vi "SeqEditor_Allseqlist-menu.vi"(8 "error in (no error)":errorcluster, 10 "String":string, 11 "NLTest in":refnum<class "NLTest.lvclass">) -> (0 "error out":errorcluster, 3 "NLTest out":refnum<class "NLTest.lvclass">)   [LabVIEW 2017, in "NLTest.lvclass"]
uses:
  NLTest.lvclass
  NLTest.lvclass/NLTest.ctl
  allseqanddata.ctl
panel:
  in  "确认":bool
  in  "新名称":string
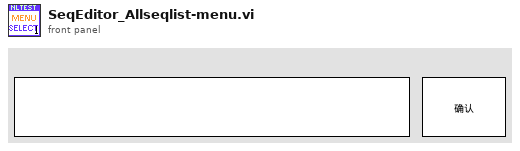
[diagram p1: front panel]
types:
  T1 = enum32{"Invalid", "Standard", "Closed", "Hidden", "Minimized", "Maximized"}
  T2 = typedef "NLTest.lvclass/allseqanddata.ctl" = cluster{"seqname":string, "seqdata":string[]}
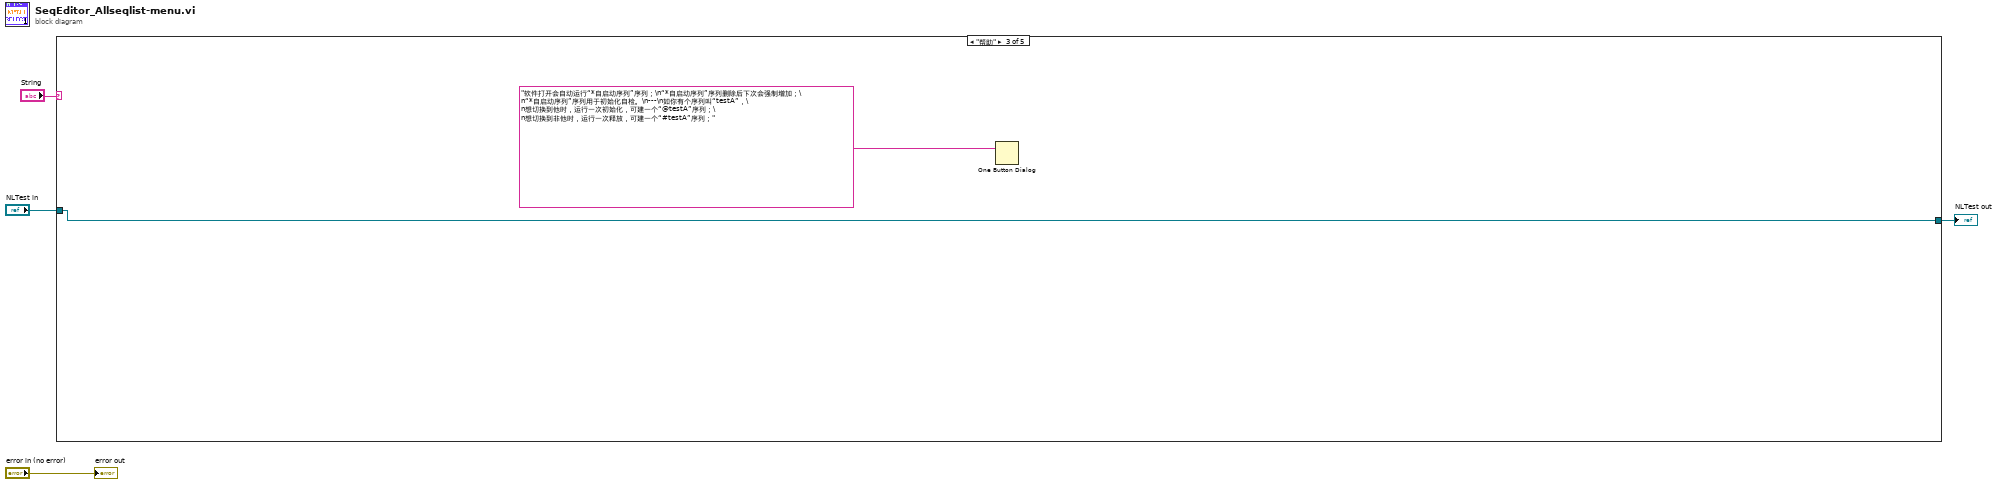
[diagram p0: block diagram]
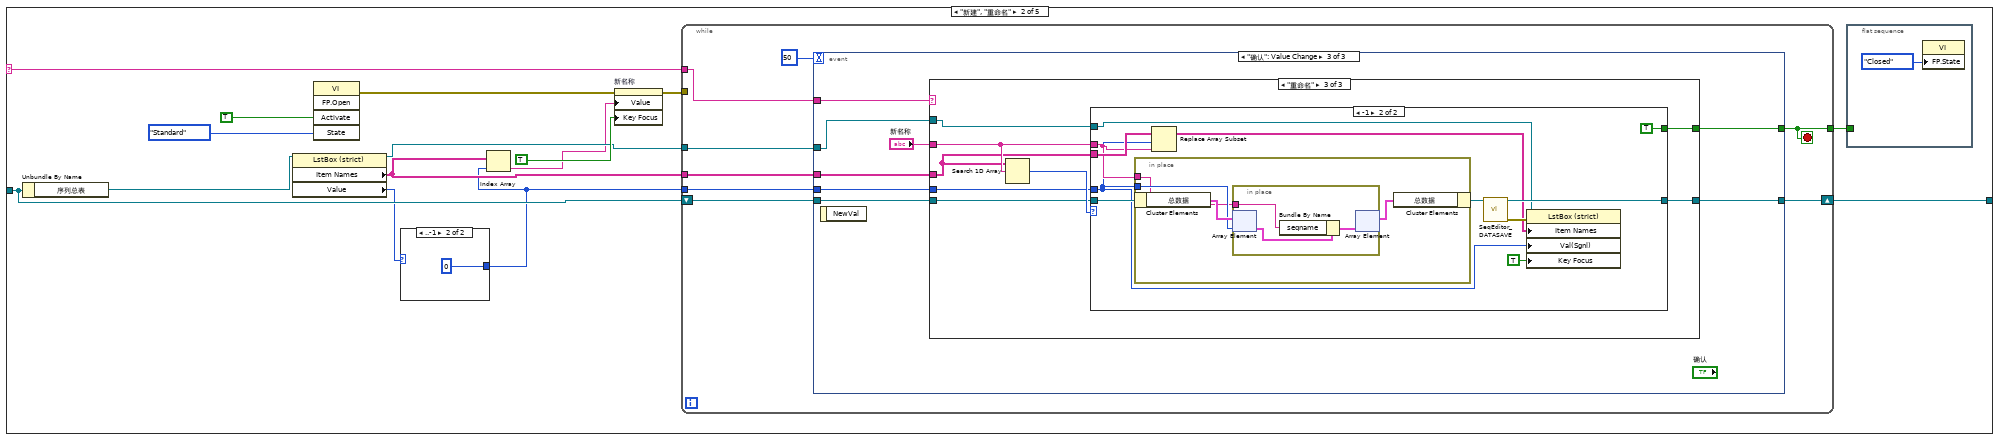
[diagram p3: hidden frame]
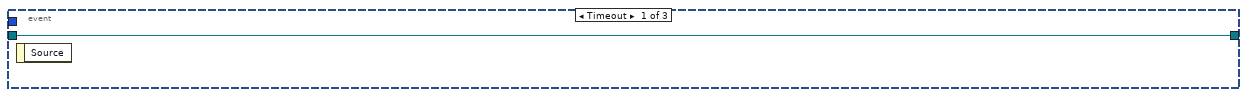
[diagram p5: hidden frame]
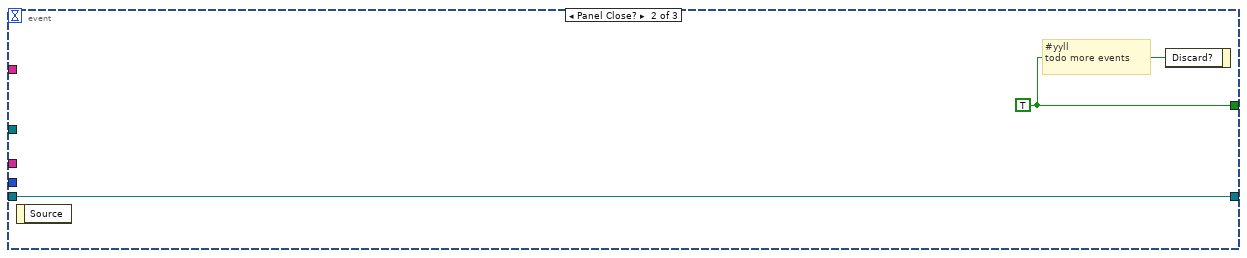
[diagram p6: hidden frame]
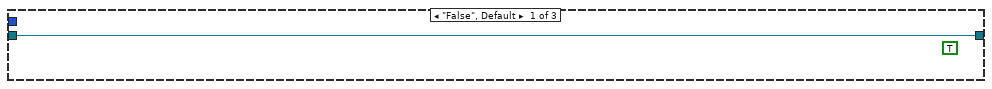
[diagram p7: hidden frame]
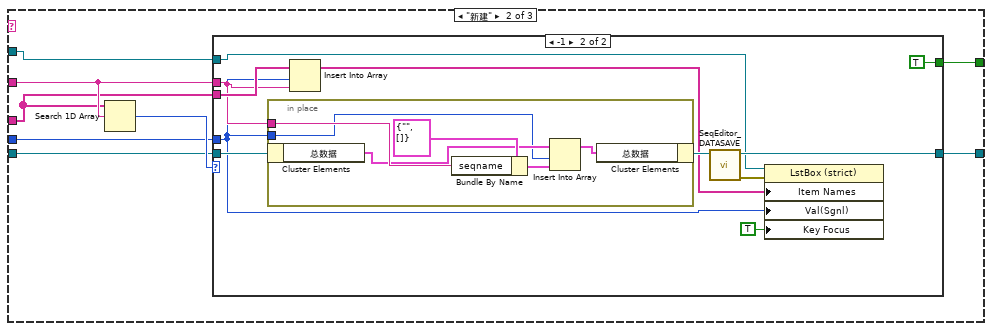
[diagram p8: hidden frame]
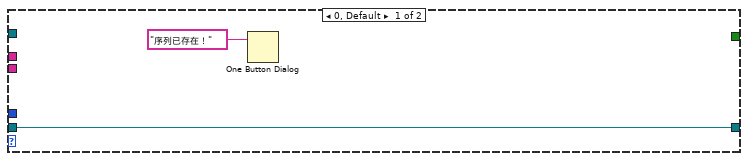
[diagram p9: hidden frame]
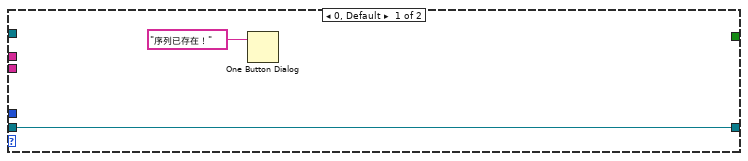
[diagram p10: hidden frame]
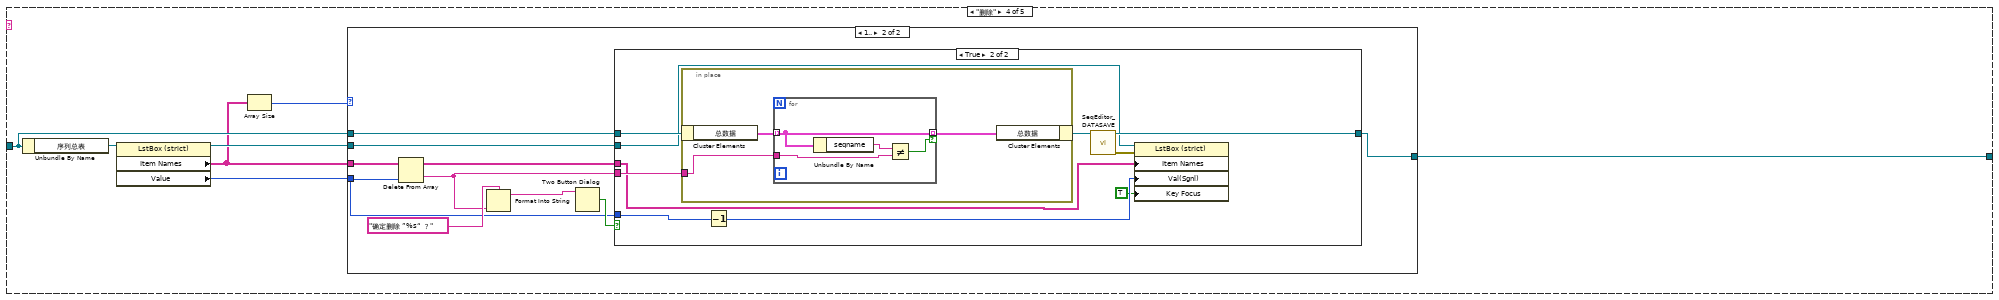
[diagram p11: hidden frame]
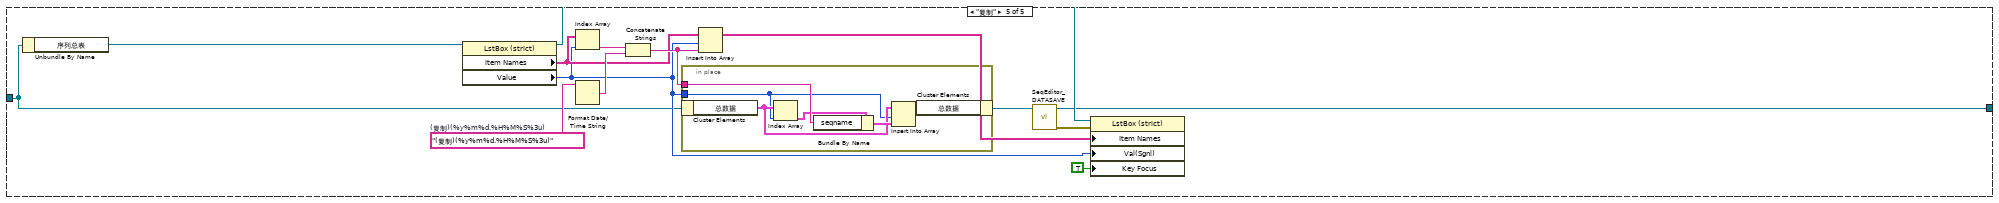
[diagram p14: hidden frame]
diagram:
  n1 = case shown="\"帮助\"" "String" {
    selector: "String" -> [_ w11 _ _ _]
    tunnel: "NLTest in" -> [w5 w14 w99 w105 w139]
    tunnel: [w5 w10 w99 w106 w138] -> w1
    frame Default {
    }
    frame "新建", "重命名" {
      n2 = Unbundle By Name(w14) -> ("序列总表"=w13:refnum<vi>)
      n3 = property class="LstBox (strict)"(reference=w13) -> (reference out=w9:refnum<vi>, "Item Names"=w12:string[], "Value"=w7:i32)  [unwired: 1 in, 1 out]
      n4 = invoke class="VI" method="FP.Open"("Activate"=TRUE ("Activate?"), "State"=T1."Standard") -> (error out=w19:errorcluster)  [unwired: 3 in, 4 out]
      n5 = case shown="..-1" w7 {
        selector: w7 -> [w21 _]
        tunnel: [w21 0] -> w6
        frame 0, Default {
        }
        frame ..-1 {
        }
      }
      n6 = Index Array(array=w12, index=w6) -> (element=w8:string)
      n7 = property on="新名称" class="Str"(error in=w19, "Value"=w8, "Key Focus"=TRUE) -> (error out=w18:errorcluster)  [unwired: 1 in, 1 out]
      n8 = while {
        tunnel: [w29] -> w15
        tunnel: w18 -> [_]
        tunnel: w11 -> [w30]
        tunnel: w12 -> [w27]
        tunnel: w9 -> [w25]
        tunnel: w6 -> [w24]
        shift-right: [w26] -> w10
        shift-left: w14 -> [w28]
        stop <- w29 stop-if-true
        n9 = event shown="[2] \"确认\": Value Change" {
          selector: _ -> [_ _ _]
          dyn-events: _ -> [_ _ _]
          timeout: 50 -> [_ _ _]
          tunnel: w30 -> [_ _ w42]
          tunnel: [_ w34 w35] -> w29
          tunnel: w28 -> [w32 w33 w41]
          tunnel: w27 -> [_ _ w39]
          tunnel: [w32 w33 w38] -> w26
          tunnel: w25 -> [_ _ w37]
          tunnel: w24 -> [_ _ w36]
          event Timeout {
            n10 = event-data() -> ()  [unwired: 1 in, 1 out]
          }
          event Panel Close? {
            w34 = TRUE ("Discard?")
            # "#yyll\ntodo more events"
            n11 = event-data() -> ()  [unwired: 1 in, 1 out]
            n12 = event-data("Discard?"=w34) -> ()  [unwired: 1 in, 1 out]
          }
          event "确认": Value Change {
            n13 = event-data() -> ()  [unwired: 1 in, 1 out]
            n14 = case shown="\"重命名\"" w42 {
              tunnel: w41 -> [w43 w50 w77]
              tunnel: "新名称" -> [_ w49 w76]
              tunnel: w39 -> [_ w46 w73]
              tunnel: [w43 w48 w75] -> w38
              tunnel: w37 -> [_ w47 w74]
              tunnel: w36 -> [_ w45 w72]
              tunnel: [_ w44 w71] -> w35
              frame "False", Default {
                (unwired) TRUE
              }
              frame "新建" {
                n15 = Search 1D Array(1D array=w46, element=w49) -> (index of element=w51:i32)  [unwired: 1 in]
                n16 = case shown="-1" w51 {
                  tunnel: w50 -> [w52 w64]
                  tunnel: w49 -> [_ w58]
                  tunnel: [w52 w62] -> w48
                  tunnel: w47 -> [_ w61]
                  tunnel: w46 -> [_ w59]
                  tunnel: w45 -> [_ w56]
                  tunnel: [_ TRUE] -> w44
                  frame 0, Default {
                    n17 = One Button Dialog(message="序列已存在！") -> ()  [unwired: 1 in, 1 out]
                  }
                  frame -1 {
                    n18 = in-place {
                      in-place-border: w58 -> [w69]
                      in-place-border: w56 -> [w67]
                      n19 = in-place-cluster #1(w64) -> ("总数据"=w68:T2[])
                      n20 = Bundle By Name(cluster=T2 {"seqname"="", "seqdata"=[]} ("allseqanddata"), "seqname"=w69) -> (w66:T2)
                      n21 = Insert Into Array(array=w68, index=w67, new element=w66) -> (w65:T2[])
                      n22 = in-place-cluster #1("总数据"=w65) -> (w63:refnum<class "NLTest.lvclass">)
                    }
                    n23 = Insert Into Array(array=w59, index=w56, new element=w58) -> (w57:string[])
                    n24 = call "SeqEditor_DATASAVE.vi"("NLTest in"=w63) -> ("error out"=w60:errorcluster, "NLTest out"=w62:refnum<class "NLTest.lvclass">)  [unwired: 9 in]
                    n25 = property class="LstBox (strict)"(reference=w61, error in=w60, "Item Names"=w57, "Val(Sgnl)"=w56, "Key Focus"=TRUE) -> ()  [unwired: 2 out]
                  }
                }
              }
              frame "重命名" {
                n26 = Search 1D Array(1D array=w73, element=w76) -> (index of element=w78:i32)  [unwired: 1 in]
                n27 = case shown="-1" w78 {
                  tunnel: w77 -> [w79 w91]
                  tunnel: w76 -> [_ w85]
                  tunnel: [w79 w89] -> w75
                  tunnel: w74 -> [_ w88]
                  tunnel: w73 -> [_ w86]
                  tunnel: w72 -> [_ w83]
                  tunnel: [_ TRUE] -> w71
                  frame 0, Default {
                    n28 = One Button Dialog(message="序列已存在！") -> ()  [unwired: 1 in, 1 out]
                  }
                  frame -1 {
                    n29 = in-place {
                      in-place-border: w85 -> [w93]
                      in-place-border: w83 -> [w94]
                      n30 = in-place-cluster #2(w91) -> ("总数据"=w95:T2[])
                      n31 = in-place {
                        in-place-border: w93 -> [w96]
                        n32 = in-place-array #3(w95, w94) -> (w98:T2)
                        n33 = Bundle By Name(cluster=w98, "seqname"=w96) -> (w97:T2)
                        n34 = in-place-array #3(w97) -> (w92:T2[])  [unwired: 1 out]
                      }
                      n35 = in-place-cluster #2("总数据"=w92) -> (w90:refnum<class "NLTest.lvclass">)
                    }
                    n36 = Replace Array Subset(array=w86, new element=w85, index=w83) -> (w84:string[])
                    n37 = call "SeqEditor_DATASAVE.vi"("NLTest in"=w90) -> ("error out"=w87:errorcluster, "NLTest out"=w89:refnum<class "NLTest.lvclass">)  [unwired: 9 in]
                    n38 = property class="LstBox (strict)"(reference=w88, error in=w87, "Item Names"=w84, "Val(Sgnl)"=w83, "Key Focus"=TRUE) -> ()  [unwired: 2 out]
                  }
                }
              }
            }
          }
        }
      }
      n39 = flat-sequence {
        tunnel: w15 -> [_]
        frame #0 {
          n40 = property class="VI"("FP.State"=T1."Closed" ("前面板窗口:状态")) -> ()  [unwired: 2 in, 2 out]
        }
      }
    }
    frame "帮助" {
      n41 = One Button Dialog(message="软件打开会自动运行“*自启动序列”序列；\n“*自启动序列”序列删除后下次会强制增加；\n“*自启动序列”序列用于初始化自检。\n---\n如你有个序列叫“testA”，\n想切换到他时，运行一次初始化，可建一个“@testA”序列；\n想切换到非他时，运行一次释放，可建一个“#testA”序列；") -> ()  [unwired: 1 in, 1 out]
    }
    frame "删除" {
      n42 = Unbundle By Name(w105) -> ("序列总表"=w107:refnum<vi>)
      n43 = property class="LstBox (strict)"(reference=w107) -> (reference out=w104:refnum<vi>, "Item Names"=w102:string[], "Value"=w103:i32)  [unwired: 1 in, 1 out]
      n44 = Array Size(array=w102) -> (size(s)=w101:i32)
      n45 = case shown="1.." w101 {
        tunnel: [w108 w115] -> w106
        tunnel: w105 -> [w108 w114]
        tunnel: w104 -> [_ w112]
        tunnel: w103 -> [_ w110]
        tunnel: w102 -> [_ w109]
        frame 0, Default {
        }
        frame 1.. {
          n46 = Delete From Array(array=w109, index=w110) -> (deleted portion=w113:string, array with subset deleted=w111:string[])  [unwired: 1 in]
          n47 = Format Into String(format string="确定删除 ”%s“ ？" ("message"), w113) -> (resulting string=w116:string)  [unwired: 2 in, 1 out]
          n48 = Two Button Dialog(message=w116) -> (T button?=w118:bool)  [unwired: 2 in]
          n49 = case shown="True" w118 {
            tunnel: [w119 w126] -> w115
            tunnel: w114 -> [w119 w128]
            tunnel: w113 -> [_ w129]
            tunnel: w112 -> [_ w125]
            tunnel: w111 -> [_ w124]
            tunnel: w110 -> [_ w123]
            frame False {
            }
            frame True {
              n50 = in-place {
                in-place-border: w129 -> [w132]
                n51 = in-place-cluster #4(w128) -> ("总数据"=w131:T2[])
                n52 = for {
                  tunnel: w131 -> [w134] mode=indexing
                  tunnel: w132 -> [w135]
                  tunnel: [w134] -> w130 mode=indexing if=w133
                  n53 = Unbundle By Name(w134) -> ("seqname"=w136:string)
                  n54 = Not Equal?(x=w136, y=w135) -> (x != y?=w133:bool)
                }
                n55 = in-place-cluster #4("总数据"=w130) -> (w127:refnum<class "NLTest.lvclass">)
              }
              n56 = Decrement(x=w123) -> (x-1=w122:i32)
              n57 = call "SeqEditor_DATASAVE.vi"("NLTest in"=w127) -> ("error out"=w121:errorcluster, "NLTest out"=w126:refnum<class "NLTest.lvclass">)  [unwired: 9 in]
              n58 = property class="LstBox (strict)"(reference=w125, error in=w121, "Item Names"=w124, "Val(Sgnl)"=w122, "Key Focus"=TRUE) -> ()  [unwired: 2 out]
            }
          }
        }
      }
    }
    frame "复制" {
      w147 = "(复制)(%y%m%d.%H%M%S%3u)"  # (复制)(%y%m%d.%H%M%S%3u)
      n59 = Unbundle By Name(w139) -> ("序列总表"=w144:refnum<vi>)
      n60 = property class="LstBox (strict)"(reference=w144) -> (reference out=w143:refnum<vi>, "Item Names"=w141:string[], "Value"=w140:i32)  [unwired: 1 in, 1 out]
      n61 = Index Array(array=w141, index=w140) -> (element=w142:string)
      n62 = Format Date/Time String(time format string (%c)=w147) -> (date/time string=w146:string)  [unwired: 2 in]
      n63 = Concatenate Strings(w142, w146) -> (w145:string)
      n64 = in-place {
        in-place-border: w145 -> [w156]
        in-place-border: w140 -> [w152]
        n65 = in-place-cluster #5(w139) -> ("总数据"=w153:T2[])
        n66 = Index Array(array=w153, index=w152) -> (element=w151:T2)
        n67 = Bundle By Name(cluster=w151, "seqname"=w156) -> (w155:T2)
        n68 = Insert Into Array(array=w153, index=w152, new element=w155) -> (w154:T2[])
        n69 = in-place-cluster #5("总数据"=w154) -> (w150:refnum<class "NLTest.lvclass">)
      }
      n70 = Insert Into Array(array=w141, index=w140, new element=w145) -> (w148:string[])
      n71 = call "SeqEditor_DATASAVE.vi"("NLTest in"=w150) -> ("error out"=w149:errorcluster, "NLTest out"=w138:refnum<class "NLTest.lvclass">)  [unwired: 9 in]
      n72 = property class="LstBox (strict)"(reference=w143, error in=w149, "Item Names"=w148, "Val(Sgnl)"=w140, "Key Focus"=TRUE) -> ()  [unwired: 2 out]
    }
  }
  "NLTest out" <- w1
  "error out" <- "error in (no error)"
